vi "VM3 - Write Variables (ANY).vi"(6 "atomic (F)":bool, 7 "VC Handle":T4, 8 "error in":errorcluster, 9 "writer IDs":u32[](array[numeric]), 10 "values in":T2(array[cluster]), 11 "name_specs":string[](array[string])) -> (0 "error out":errorcluster, 1 "stats":T1[](array[typedef]), 3 "dup name_specs":string[](array[string]), 4 "errCodes":T3[](array[typedef]) items=["No error", "Invalid variable type", "Variable not found", "Variable already exists", "Invalid context handle", "Input error", "Invalid data format", "No history attached", "History already attached", "Invalid history parameters", "Wrong variable name", "Wrong alias name", "Non-unique alias", "Alias not found", "No alias associated", "Alias already associated", "Wrong context name", "Non-unique context name", "Context name not found", "Invalid parameter", "Generic error", "Memory Full", "Unrecognized LV error", "Unknown error code"])   [LabVIEW 2021]
doc: "This VI writes to multiple variables of arbitrary data types; both predefined and user-defined data types are supported. Refer to the VI Help for more details.\n\n<b>VC Handle</b> specifies the handle of the variable context. To operate on a global variable, pass -1 to this input. \n<b>name_specs</b> defines the name specifiers of the target variables; usually, a name specifier is merely a variable name (see the VI Help for more options).\n\n<b>values in</b> specifies the variable values to be written. This array must have the same size as <b>name_specs</b>. Each element of this array is a cluster with three members:\n (1) <b>datatype</b> defines the data type code.\n (2) <b>DBL</b> specifies a variable value of the <b>DBL Number</b> type.\n (3) <b>STR</b> specifies a variable value for all other data types. This value must be represented in the Flattened-To-String format, with the exception of the <b>String</b> data type.\n\n<b>writer IDs</b> specifies the Writer IDs for the respective elements in <b>name_specs</b> and <b>values</b>. If the size of this array is less than the size of <b>name_specs</b>, its first element is bound to all values.\n\n<b>atomic (F)</b>, if TRUE, guarantees that all variables are written in an atomic transaction. This prevents other VIs or threads from modifying the variables during execution.\n\n<b>stats</b> returns additional information about the variable values, such as their Writer ID, update time, and update counter.\n\n<b>errCodes</b> returns VarMan error codes individually for each variable. If any element in this array is non-zero, the <b>error out</b> cluster returns the corresponding error.\n\n::: CalcExpress Toolkit :::\nCopyright (c) 2000-2026 Konstantin Shifershteyn. All rights reserved."
uses:
  cetypes.llb/VarMan Variable Context Handle.ctl
  cetypes.llb/VarMan Error Code.ctl
  cetypes.llb/VarMan Variable Data Statistics.ctl
  <vilib>/Utility/error.llb/Error Cluster From Error Code.vi
  <vilib>/ErrorRing/Error Ring.xnode
  cersrc/celveng32.dll
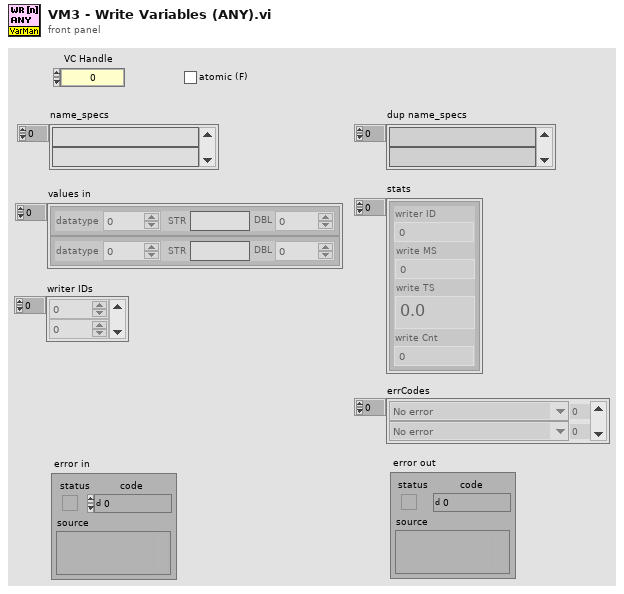
[diagram p1: front panel]
types:
  T1 = typedef "VarMan Variable Data Statistics.ctl" = cluster{"writer ID":u32, "write MS":u32, "write TS":dbl, "write Cnt":u32}
  T2 = cluster{"datatype":u32, "STR":string, "DBL":dbl}[]
  T3 = typedef "VarMan Error Code.ctl" = u16
  T4 = typedef "VarMan Variable Context Handle.ctl" = i32
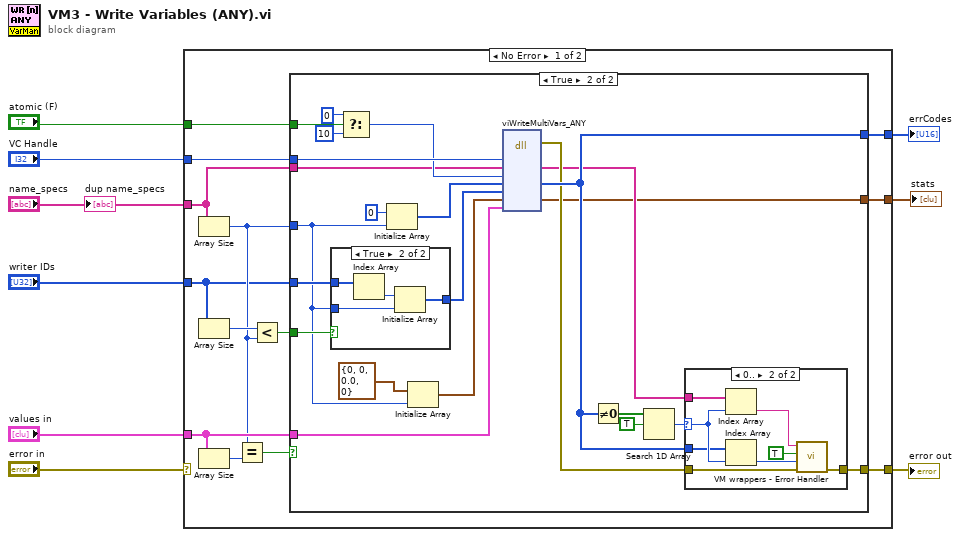
[diagram p0: block diagram]
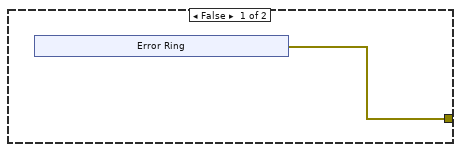
[diagram p2: hidden frame]
diagram:
  n1 = case shown="No Error" "error in" {
    selector: "error in" -> [_ w65]
    tunnel: [w18 w65] -> w8
    tunnel: "VC Handle" -> [w22 _]
    tunnel: "name_specs" -> [w19 _]
    tunnel: "atomic (F)" -> [w21 _]
    tunnel: [w20 _] -> w5
    tunnel: "values in" -> [w17 _]
    tunnel: "writer IDs" -> [w12 _]
    tunnel: [w10 _] -> w1
    frame No Error {
      n2 = Array Size(array=w19) -> (size(s)=w13:i32)
      n3 = Array Size(array=w12) -> (size(s)=w14:i32)
      n4 = Array Size(array=w17) -> (size(s)=w16:i32)
      n5 = Equal?(x=w13, y=w16) -> (x = y?=w15:bool)
      n6 = Less?(x=w14, y=w13) -> (x < y?=w11:bool)
      n7 = case shown="True" w15 {
        tunnel: w22 -> [_ w50]
        tunnel: w21 -> [_ w48]
        tunnel: [_ w43] -> w20
        tunnel: w19 -> [_ w42]
        tunnel: [w23 w40] -> w18
        tunnel: w17 -> [_ w36]
        tunnel: w13 -> [_ w30]
        tunnel: w12 -> [_ w34]
        tunnel: w11 -> [_ w32]
        tunnel: [_ w28] -> w10
        frame False {
          n8 = xnode "Error Ring"() -> ("error out"=w23:errorcluster)
        }
        frame True {
          n9 = case shown="True" w32 {
            tunnel: [w51 w53] -> w33
            tunnel: w34 -> [w51 w55]
            tunnel: w30 -> [_ w52]
            frame False {
            }
            frame True {
              n10 = Index Array(array=w55) -> (element=w54:u32)  [unwired: 1 in]
              n11 = Initialize Array(w54, w52) -> (w53:u32[])
            }
          }
          n12 = Select(t=0, s=w48, f=10) -> (s? t:f=w46:i32)
          n13 = Initialize Array(u16 0 ("element"), w30) -> (w44:u16[])
          n14 = Initialize Array(T1 {"writer ID"=0, "write MS"=0, "write TS"=0.0, "write Cnt"=0} ("stats"), w30) -> (w29:T1[])
          n15 = dll-call lib="C:/LV Projects/CalcExpress 40 LV2021/vi.lib/addons/CalcExpress/cersrc/celveng*.dll" fn="viWriteMultiVars_ANY"("vch"=w50, "names"=w42, "lock_cycle"=w46, "errCodes"=w44, "writerIDs"=w33, "wrStats"=w29, "values"=w36) -> (error out=w41:errorcluster, "names"=w35:string[], "errCodes"=w43:u16[], "wrStats"=w28:T1[])  [unwired: 8 in, 1 out]
          n16 = Not Equal To 0?(x=w43) -> (x != 0?=w39:bool[])
          n17 = Search 1D Array(1D array=w39, element=TRUE) -> (index of element=w37:i32)  [unwired: 1 in]
          n18 = case shown="0.." w37 {
            selector: w37 -> [_ w64]
            tunnel: w43 -> [_ w63]
            tunnel: w35 -> [_ w60]
            tunnel: w41 -> [w56 w58]
            tunnel: [w56 w57] -> w40
            frame ..-1 {
            }
            frame 0.. {
              n19 = Index Array(array=w60, index=w64) -> (element=w59:string)
              n20 = Index Array(array=w63, index=w64) -> (element=w62:u16)
              n21 = call "VM wrappers - Error Handler.vi"("error before"=w58, "VarMan error"=w62, "show name spec (F)"=TRUE, "name spec"=w59) -> ("error out"=w57:errorcluster)  [unwired: 6 in, 1 out]
            }
          }
        }
      }
    }
    frame Error {
    }
  }
  "error out" <- w8
  "errCodes" <- w5
  "stats" <- w1
  "dup name_specs" <- "name_specs"
